vi "Arreglo_Unidimensional.vi"() -> ()   [LabVIEW 2026]
panel:
  in  "NUEVO VALOR":dbl
  in  "INDICE":u16
  out "INDICADOR":dbl[](array[numeric])
  in  "ORIGINAL":dbl[](array[numeric])
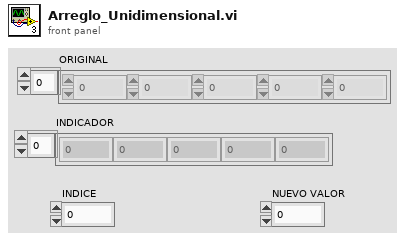
[diagram p1: front panel]
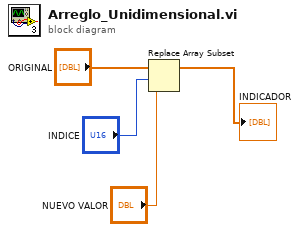
[diagram p0: block diagram]
diagram:
  n1 = Replace Array Subset(array="ORIGINAL", new element="NUEVO VALOR", index="INDICE") -> (→"INDICADOR":dbl[])
